vi "Timeout Manager.vi"(8 "error in (no error)":errorcluster, 11 "bt_WaitOn_Synch in":refnum<class "bt_WaitOn_Synch.lvclass">) -> (0 "error out":errorcluster, 1 "Timeout":i32, 2 "Timeout Now?":bool, 3 "bt_WaitOn_Synch out":refnum<class "bt_WaitOn_Synch.lvclass">, 4 "First Time":bool)   [LabVIEW 2021, in "BT.lvlib" / "bt_WaitOn_Synch.lvclass"]
uses:
  bt_WaitOn_Synch.lvclass
  bt_WaitOn_Synch.lvclass/bt_WaitOn_Synch.ctl
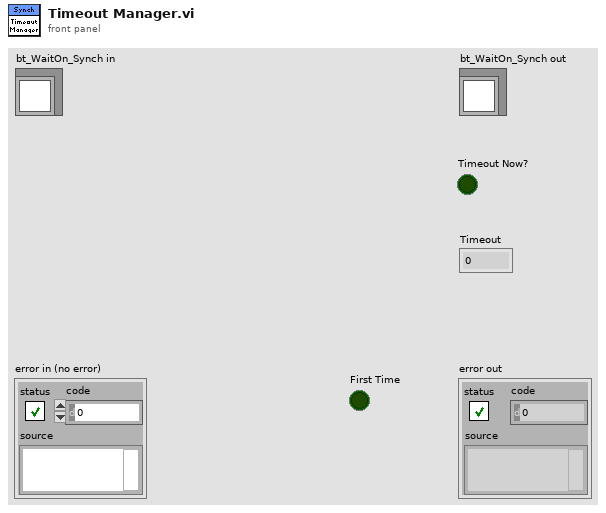
[diagram p1: front panel]
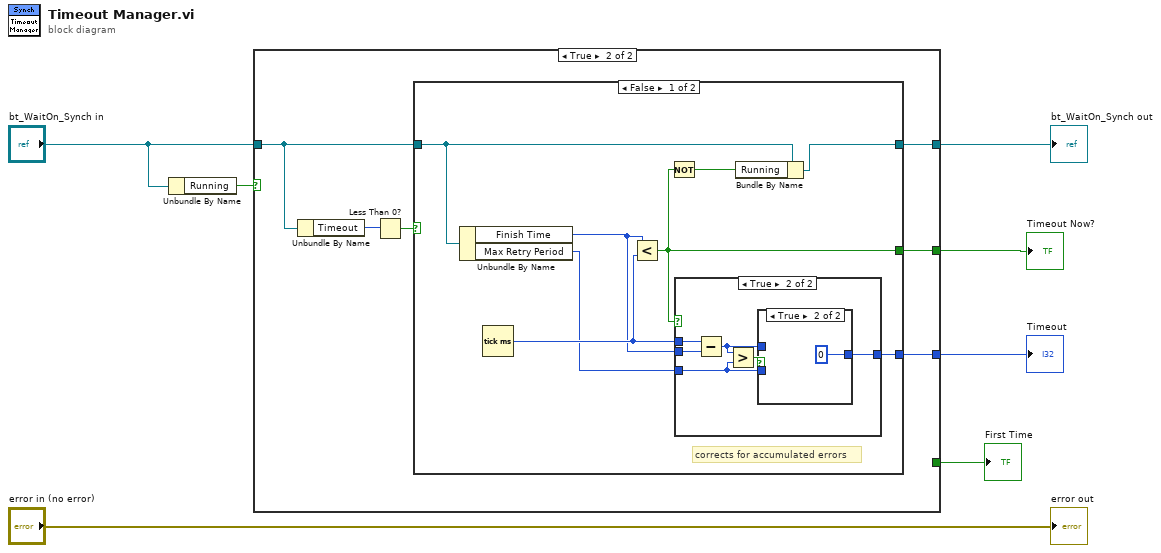
[diagram p0: block diagram]
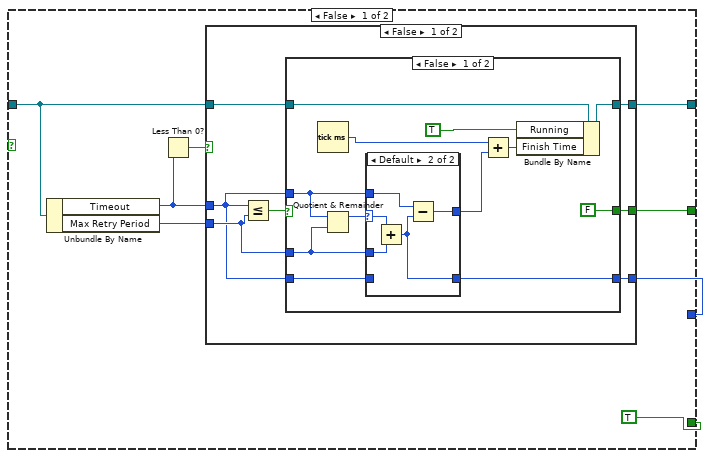
[diagram p2: hidden frame]
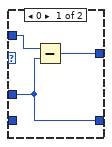
[diagram p3: hidden frame]
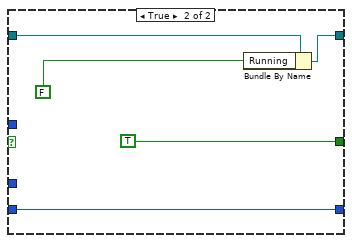
[diagram p4: hidden frame]
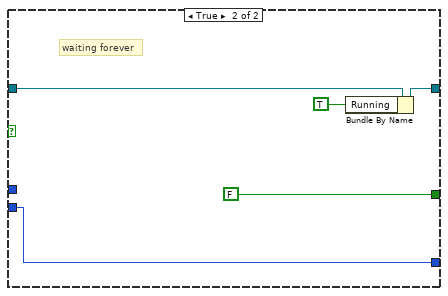
[diagram p5: hidden frame]
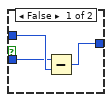
[diagram p7: hidden frame]
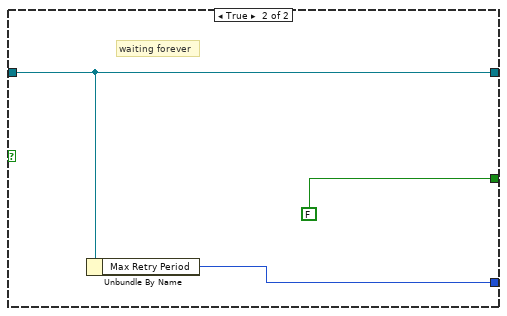
[diagram p8: hidden frame]
diagram:
  n1 = Unbundle By Name("bt_WaitOn_Synch in") -> ("Running"=w6:bool)
  n2 = case shown="True" w6 {
    tunnel: "bt_WaitOn_Synch in" -> [w14 w56]
    tunnel: [w15 w55] -> w4
    tunnel: [w13 w54] -> w3
    tunnel: [w12 w53] -> w2
    tunnel: [TRUE _] -> w1
    frame False {
      n3 = Unbundle By Name(w14) -> ("Timeout"=w9:i32, "Max Retry Period"=w11:i32)
      n4 = Less Than 0?(x=w9) -> (x < 0?=w10:bool)
      n5 = case shown="False" w10 {
        tunnel: [w22 w49] -> w15
        tunnel: w14 -> [w21 w52]
        tunnel: [w19 FALSE] -> w13
        tunnel: [w18 w50] -> w12
        tunnel: w9 -> [w16 _]
        tunnel: w11 -> [w17 w50]
        frame False {
          n6 = Less Or Equal?(x=w16, y=w17) -> (x <= y?=w20:bool)
          n7 = case shown="False" w20 {
            tunnel: [w33 w47] -> w22
            tunnel: w21 -> [w34 w46]
            tunnel: [FALSE TRUE] -> w19
            tunnel: [w27 w43] -> w18
            tunnel: w16 -> [w26 w43]
            tunnel: w17 -> [w25 _]
            tunnel: w16 -> [w24 _]
            frame False {
              n8 = Tick Count (ms)() -> (millisecond timer value=w30:u32)
              n9 = Quotient & Remainder(x=w24, y=w25) -> (x-y*floor(x/y)=w28:i32)  [unwired: 1 out]
              n10 = case shown="Default" w28 {
                selector: w28 -> [_ w40]
                tunnel: [w36 w38] -> w27
                tunnel: w26 -> [_ _]
                tunnel: w25 -> [w36 w39]
                tunnel: w24 -> [w37 w41]
                tunnel: [w35 w42] -> w23
                frame 0 {
                  n11 = Subtract(x=w37, y=w36) -> (x-y=w35:i32)
                }
                frame Default {
                  n12 = Add(x=w40, y=w39) -> (x+y=w38:i32)
                  n13 = Subtract(x=w41, y=w38) -> (x-y=w42:i32)
                }
              }
              n14 = Add(x=w30, y=w23) -> (x+y=w29:u32)
              n15 = Bundle By Name(cluster=w34, "Running"=TRUE, "Finish Time"=w29) -> (w33:refnum<class "bt_WaitOn_Synch.lvclass">)
            }
            frame True {
              n16 = Bundle By Name(cluster=w46, "Running"=FALSE) -> (w47:refnum<class "bt_WaitOn_Synch.lvclass">)
            }
          }
        }
        frame True {
          # "waiting forever"
          n17 = Bundle By Name(cluster=w52, "Running"=TRUE) -> (w49:refnum<class "bt_WaitOn_Synch.lvclass">)
        }
      }
    }
    frame True {
      n18 = Unbundle By Name(w56) -> ("Timeout"=w58:i32)
      n19 = Less Than 0?(x=w58) -> (x < 0?=w57:bool)
      n20 = case shown="False" w57 {
        tunnel: w56 -> [w66 w80]
        tunnel: [w65 w80] -> w55
        tunnel: [w63 FALSE] -> w54
        tunnel: [w59 w78] -> w53
        frame False {
          # "corrects for accumulated errors"
          n21 = Unbundle By Name(w66) -> ("Finish Time"=w61:u32, "Max Retry Period"=w60:i32)
          n22 = Tick Count (ms)() -> (millisecond timer value=w62:u32)
          n23 = Less?(x=w61, y=w62) -> (x < y?=w63:bool)
          n24 = Not(x=w63) -> (.not. x?=w64:bool)
          n25 = case shown="True" w63 {
            tunnel: w62 -> [_ w73]
            tunnel: w61 -> [_ w72]
            tunnel: w60 -> [w67 w70]
            tunnel: [w67 w71] -> w59
            frame False {
            }
            frame True {
              n26 = Subtract(x=w73, y=w72) -> (x-y=w69:u32)
              n27 = Greater?(x=w69, y=w70) -> (0:w68:bool)
              n28 = case shown="True" w68 {
                tunnel: w69 -> [w76 _]
                tunnel: w70 -> [w75 _]
                tunnel: [w74 u32 0] -> w71
                frame False {
                  n29 = Subtract(x=w75, y=w76) -> (x-y=w74:u32)
                }
                frame True {
                }
              }
            }
          }
          n30 = Bundle By Name(cluster=w66, "Running"=w64) -> (w65:refnum<class "bt_WaitOn_Synch.lvclass">)
        }
        frame True {
          # "waiting forever"
          n31 = Unbundle By Name(w80) -> ("Max Retry Period"=w78:i32)
        }
      }
    }
  }
  "bt_WaitOn_Synch out" <- w4
  "Timeout Now?" <- w3
  "Timeout" <- w2
  "First Time" <- w1
  "error out" <- "error in (no error)"
